vi "Main.vi"() -> ()   [LabVIEW 2013]
doc: "This template is for the Queued Message Handler design pattern.\n\nThe Event Handling Loop generates messages based on user interface actions.\n\nThe Message Handling Loop processes messages generated by the Event Handling Loop, or by other messages. The messages are string values, so new messages can be added easily to the Message Cases case structure in the Message Handling Loop. Each message cluster can also provide an optional value for Message Data, which is a variant that can be converted to whatever message-specific data is required."
uses:
  <vilib>/vision/Image Controls.llb/IMAQ Image.ctl
  <vilib>/vision/Avi.llb/IMAQ AVI2 Refnum.ctl
  Image Processing/Mask ROI FG Enum.ctl
  Message Passing/MsgQ Loops enum.ctl
  System Status/Status FG Enum.ctl
  Globals/Average Sector Data.vi
  controls/UI Data.ctl
  Message Queue/Message Queue.lvlib
  User Event - Stop/User Event - Stop.lvlib
  FPGA/FPGA Frame Grabbing.lvlib
  Image Processing/Image Processing.lvlib
  Common/State Machines/State Machine Lib.lvlib
  Message Passing/Main MsgQ.lvlib
  Common/GUI/GUI.lvlib
  <vilib>/rvi/interface/nirviReadWriteControl/nirviReadWriteControl.xnode
  FGs/FPGA_Reference.ctl
  FPGA Bitfiles/WBA256SectorsSim_FPGATarget.lvbitx
  Common/Timing/Timing Lib.lvlib
  <vilib>/rvi/errors/niLvFpgaMergeErrorWithErrorCode.vi
  NiFpgaLv.dll
  <vilib>/rvi/errors/niLvFpgaAdjustHostInterfaceError.vi
panel:
  in  "Auto Acq Total":u16=400
  in  "Auto Acquire?":bool
  out "Auto Acq Count":u16=401
  out "Codec Chosen":string="Motion JPEG (NI Vision)"
  in  "Codec index":i32=4
  out "Installed Codecs":string[](array[string])=["Microsoft Video 1", "Intel IYUV codec", "Cinepak Codec by Radius", "FF Video Codec 1 (FFV1) (NI Vision)", "Motion JPEG (NI Vision)", "Y800 Uncompressed Grey Scale (NI Vision)", "YUV 4:2:0 Planar (NI Vision)"]
  out "Overlay Image":T1
  out "AVI Refnum":T2
  in  "AVI FPS":u32=200
  in  "Save to AVI?":bool
  out "Single Acq Count":u16=1
  out "Frames Acquired":u32=1
  in  "Disable Background Subtraction":bool
  out "Analysis Ticks":u32
  out "Accumulate Ticks":u32
  out "FPGA Display Image":T1(plugin-control)
  out "Right Wingbeat Avg Graph":u8[](graph)=[9, 2, 3, 6, 23, 29, 37, 22, 2, 3, 2, 2, 2, 2, 2, 2]
  in  "Start Serial Server":bool=TRUE
  out "Left Wingbeat Avg Graph":u8[](graph)=[21, 5, 10, 10, 22, 33, 35, 21, 2, 2, 2, 2, 2, 2, 1, 2]
  in  "Stop Charts":bool
  in  "Wing ROIs":T3
  out "FPGA image info":T6={"Image Type"=0, "Unit"=enum."Undefined", "X Resolution"=1200, "Y Resolution"=788, "X Step"=1.0, "Y Step"=1.0, "Image Name"="Acquired"} {"Image Type" items=["Grayscale (U8)", "Grayscale (I16)", "Grayscale (SGL)", "Complex (CSG)", "RGB (U32)", "HSL (U32)", "RGB (U64)", "Grayscale (U16)"]}
  in  "Stream?":bool
  out "FPGA Image":T1
  in  "Test Visual Response":bool
  in  "Test FPGA":bool
  out "Status Update":string="01/27/2014 11:29:43.522 :  Loading Simulation Images\r01/27/2014 11:29:43.809 :  Completed Loading Simulation Images\r01/27/2014 11:29:43.911 :  Camera Initialized\r"
  in  "Define Mask":bool
  in  "Acquire Image":bool
  in  "Stop":bool
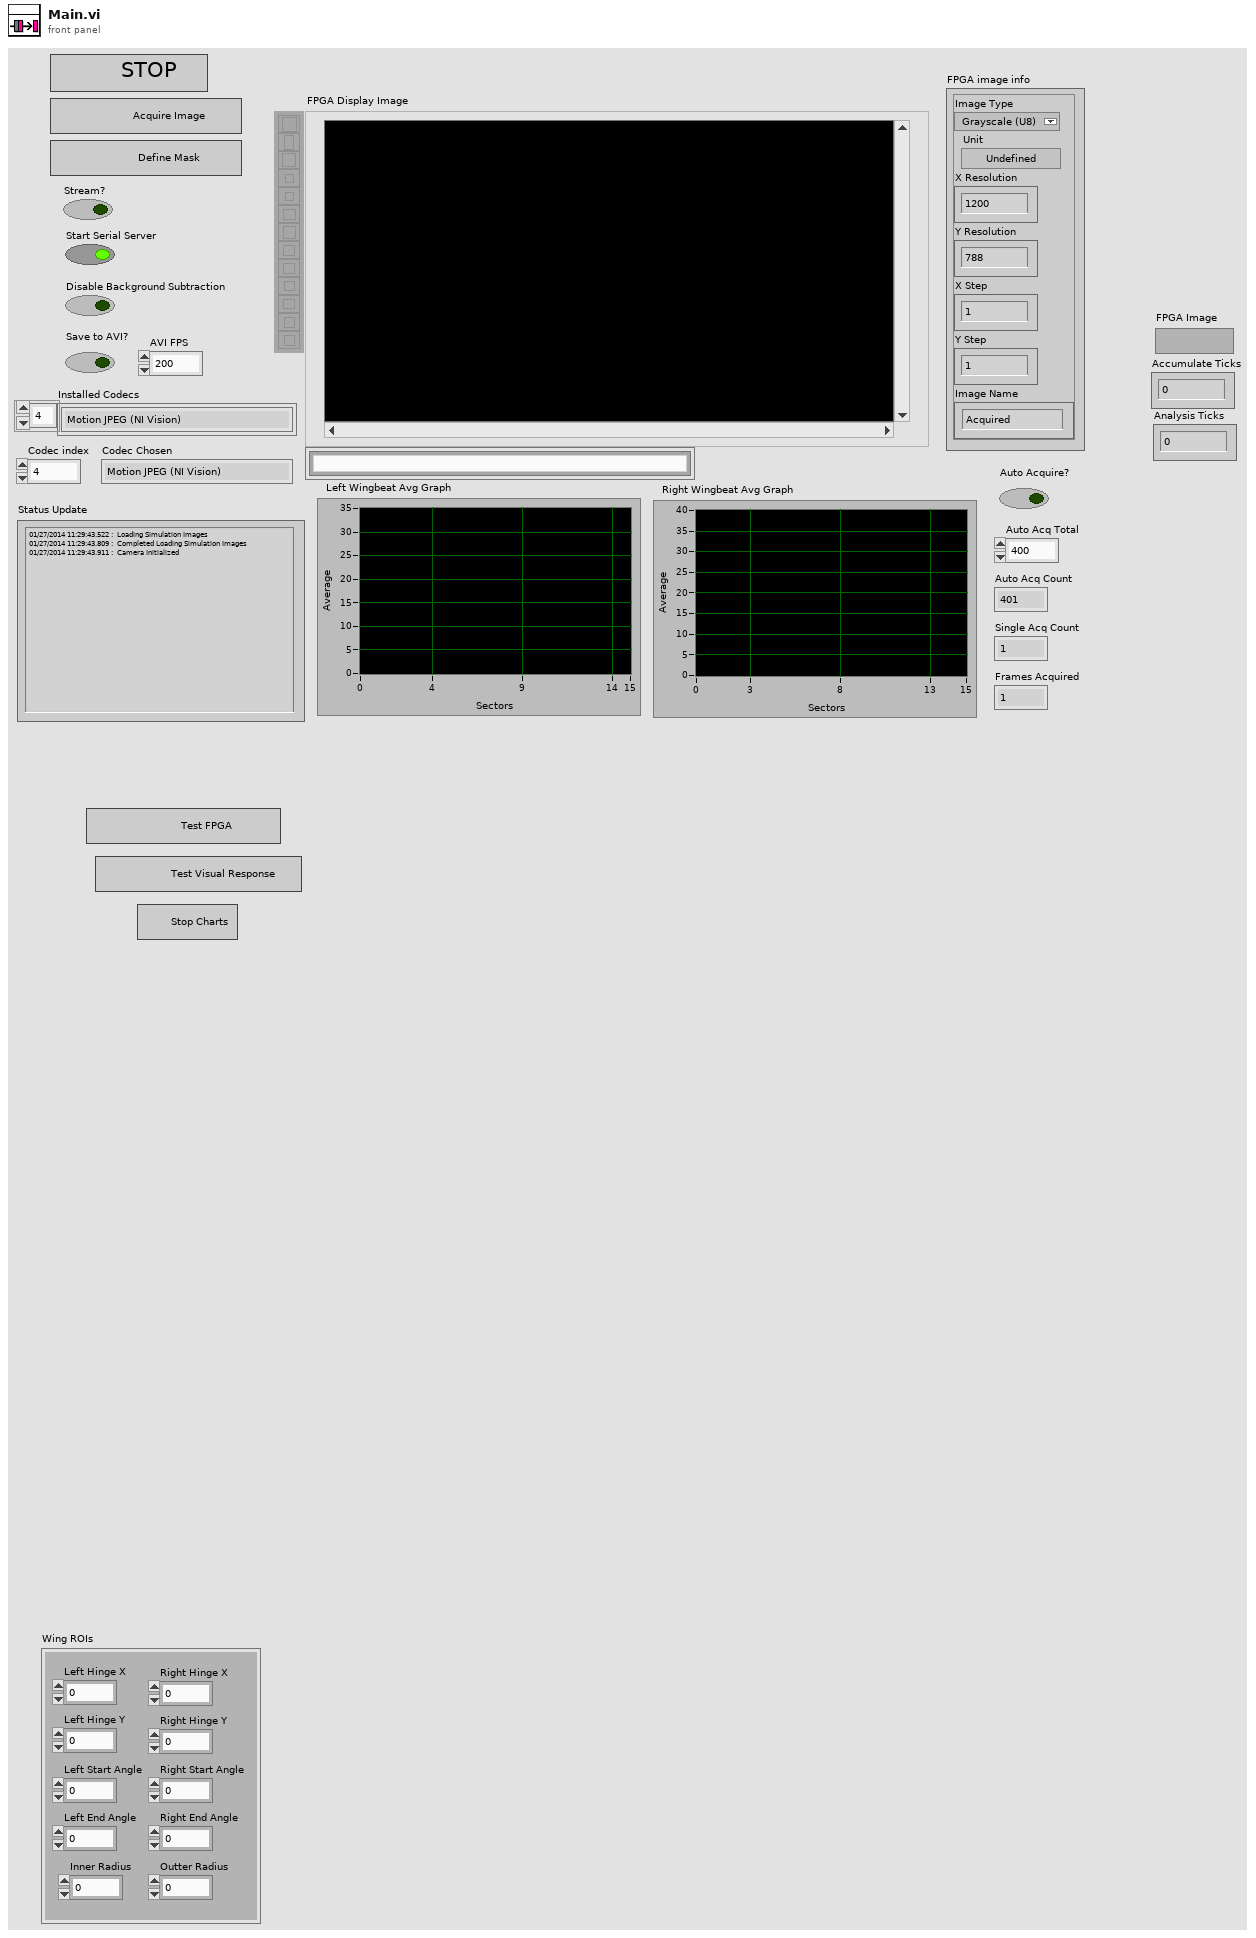
[diagram p1: front panel]
types:
  T1 = typedef "IMAQ Image.ctl" = refnum<image>
  T2 = typedef "IMAQ AVI2 Refnum.ctl" = refnum<k20>
  T3 = cluster{"Left Hinge X":u16, "Left Hinge Y":u16, "Inner Radius":u16, "Outter Radius":u16, "Right Hinge X":u16, "Right Hinge Y":u16, "Right Start Angle":i16, "Right End Angle":i16, "Left Start Angle":i16, "Left End Angle":i16}
  T4 = typedef "Image Type" = u32
  T5 = typedef "Image Unit" = enum32{"Undefined", "Angström", "Micrometer", "Millimeter", "Centimeter", "Meter", "Kilometer", "Microinch", "Inch", "Feet", "Nautical miles", "Standard miles", "Steps"}
  T6 = cluster{"Image Type":T4, "Unit":T5, "X Resolution":i32, "Y Resolution":i32, "X Step":sgl, "Y Step":sgl, "Image Name":string}
  T7 = typedef "State Machine Lib.lvlib/STATE cluster.ctl" = cluster{"State":string, "Parameters":variant}
  T8 = typedef "Main MsgQ.lvlib/MsgQ Loops enum.ctl" = enum16{"User Interface", "Image Acq"}
  T9 = typedef "Mask ROI FG Enum.ctl" = enum16{"Read", "Write", "Enable Background", "Disable Background"}
  T10 = typedef "Status FG Enum.ctl" = enum16{"Reset", "Read", "Write"}
  T11 = enum32{"Gray", "Binary", "Gradient", "Rainbow", "Temperature"}
  T12 = typedef "FPGA_Reference.ctl" = refnum<k20>
  T13 = typedef "Mask ROI Cluster.ctl" = cluster{"left annulus":T14, "right annulus":T14, "Threshold Range":cluster{"Lower value":dbl, "Upper value":dbl}, "[Avg BG]":u8[], "Number of Sectors":u8, "Left ROI":T15, "Right ROI":T15, "Left Start Angle Duty Cycle":fxp<+,8,0>, "Left End Angle Duty Cycle":fxp<+,8,0>, "Right End Angle Duty Cycle":fxp<+,8,0>, "Right Start Angle Duty Cycle":fxp<+,8,0>, "[Sector ROIs]":T15[]}
  T14 = typedef "IMAQ Circle" = cluster{"Center X":i32, "Center Y":i32, "Inner Radius":i32, "Outer Radius":i32, "Start Angle":dbl, "End Angle":dbl}
  T15 = typedef "ROI Descriptor" = cluster{"Global Rectangle":i32[], "Contours":cluster{"ID":enum32{"External", "Internal"}, "Type":u32, "Coordinates":i32[]}[]}
  T16 = typedef "UI Data.ctl" = cluster{"Boolean <Replace Me>":bool, "Initial Message":string, "Numeric <Replace Me>":dbl, "Acquire Image Ref":refnum<vi>, "Define Mask Ref":refnum<vi>, "Status Update Ref":refnum<vi>, "Stop Button Ref":refnum<vi>, "FPGA Image":T1, "Processed Image":T1, "Left Annulus":cluster{"Center X":i32, "Center Y":i32, "Inner Radius":i32, "Outer Radius":i32, "Start Angle":dbl, "End Angle":dbl}, "Right Annulus":cluster{"Center X":i32, "Center Y":i32, "Inner Radius":i32, "Outer Radius":i32, "Start Angle":dbl, "End Angle":dbl}}
  T17 = typedef "Message Queue.lvlib/All Message Queues.ctl" = cluster{"UI":refnum<queue>}
  T18 = cluster{"Center X":i32, "Center Y":i32, "Inner Radius":i32, "Outer Radius":i32, "Start Angle":dbl, "End Angle":dbl}
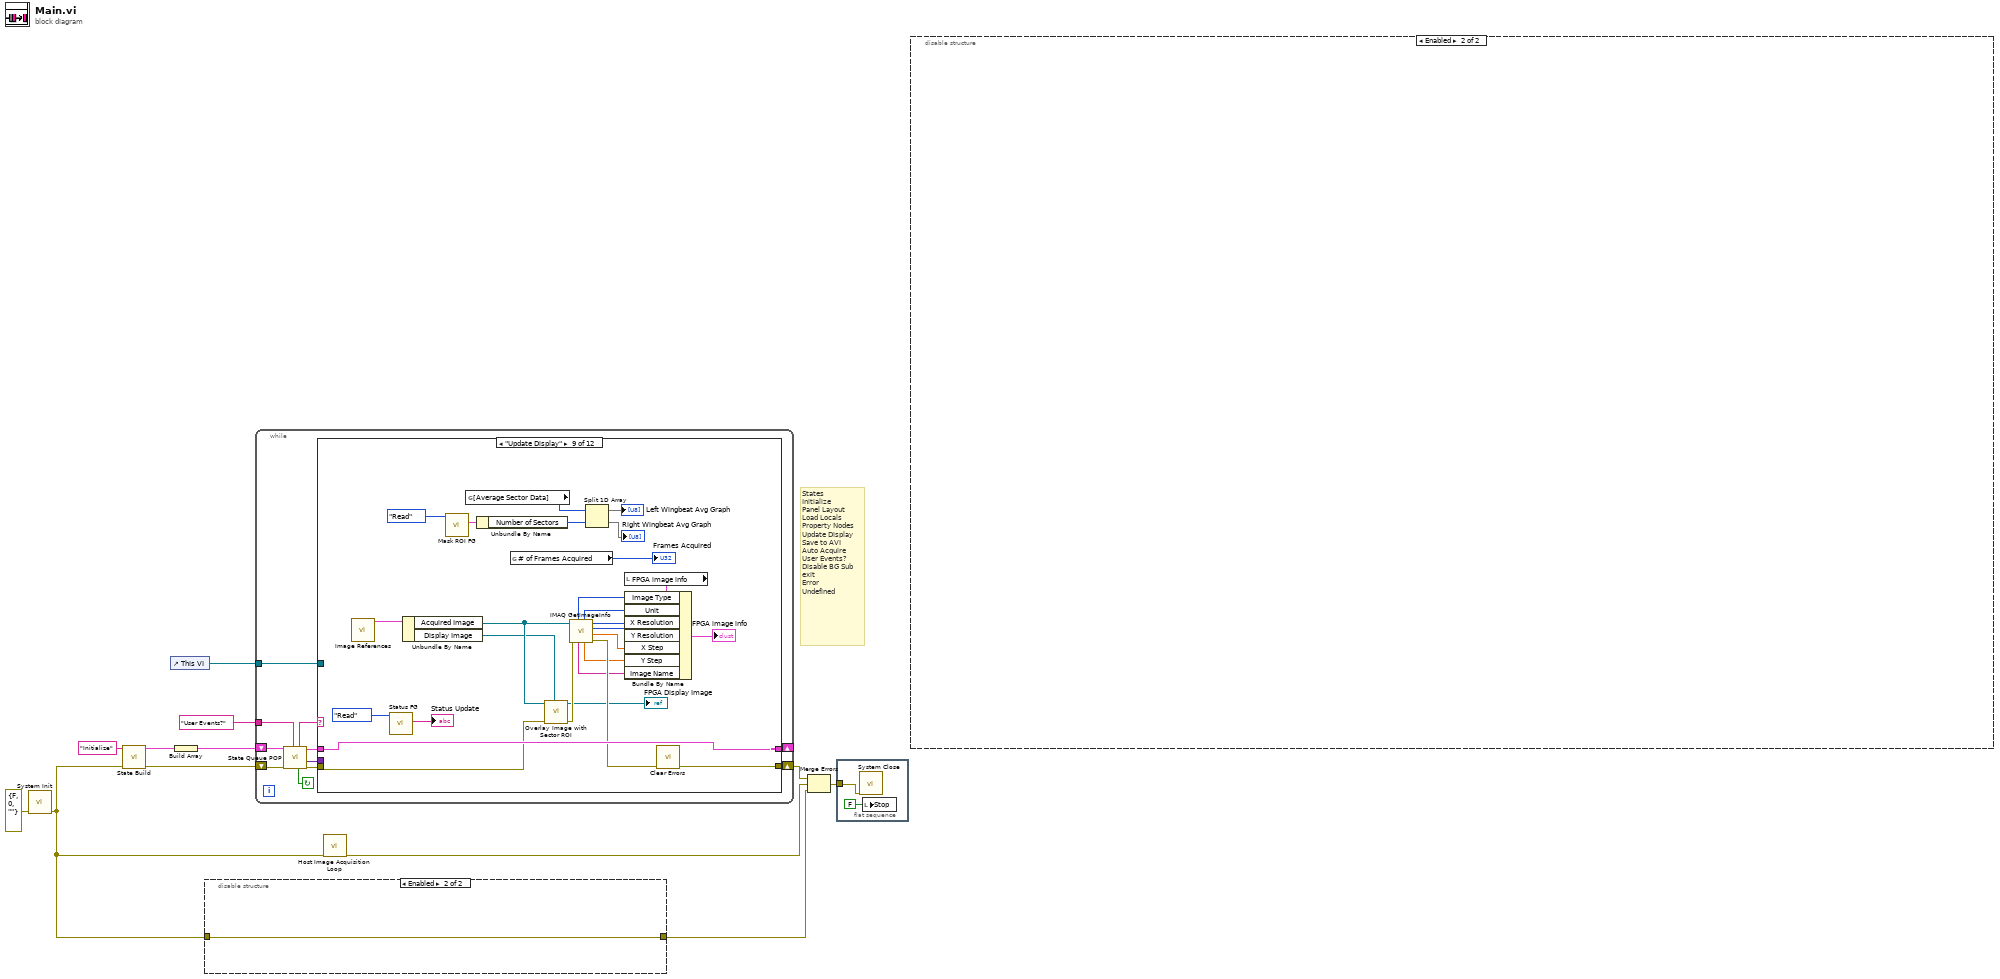
[diagram p0: block diagram]
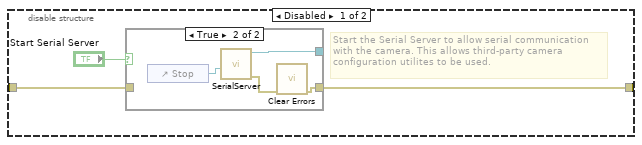
[diagram p2: hidden frame]
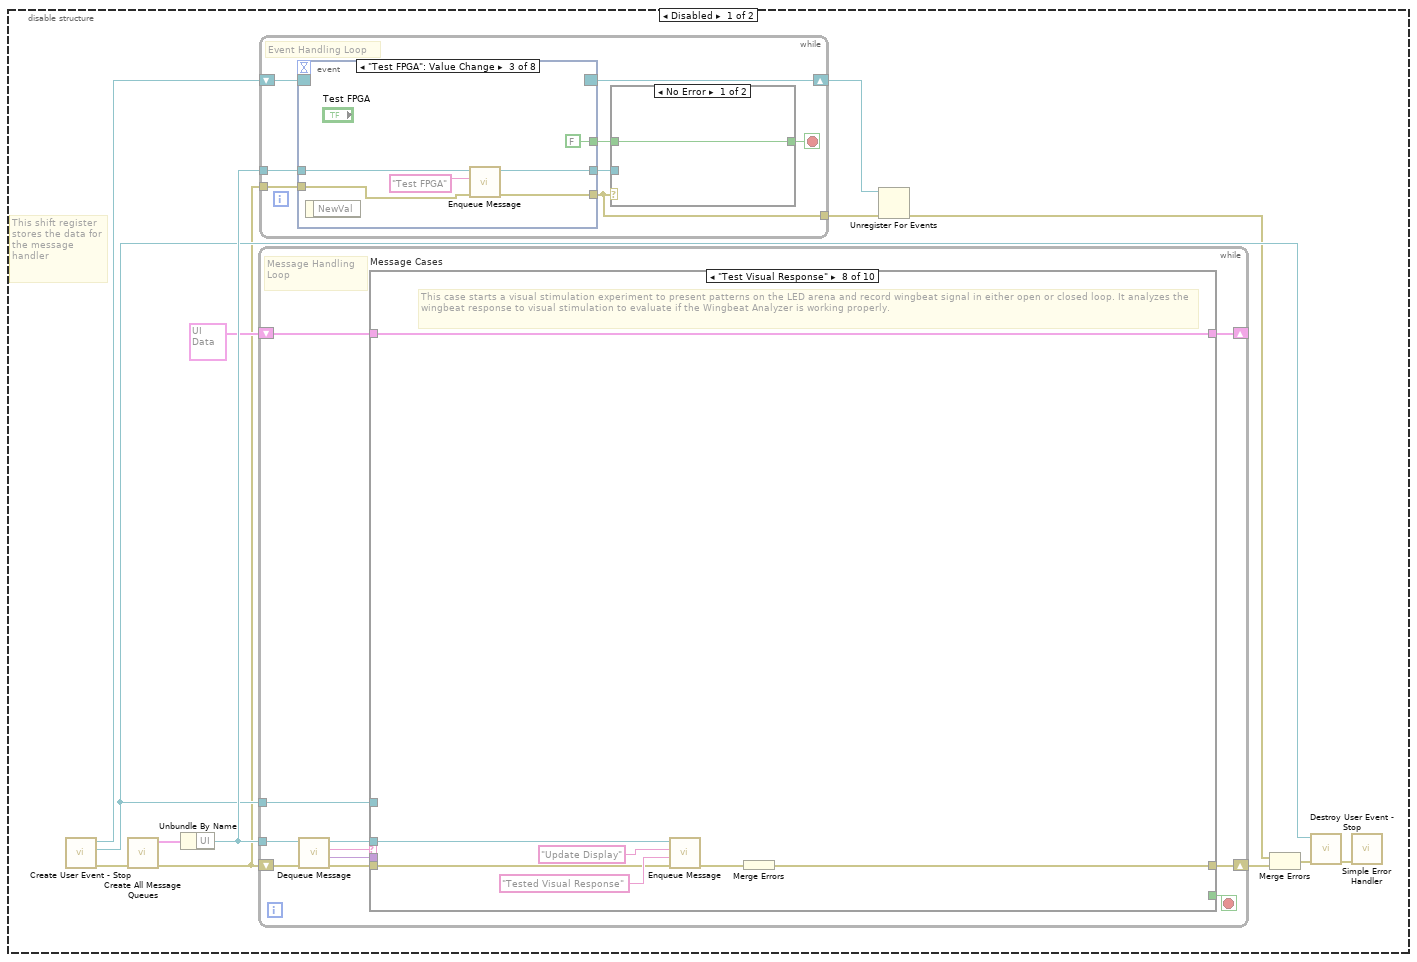
[diagram p4: hidden frame]
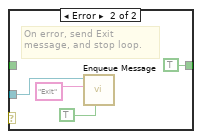
[diagram p5: hidden frame]
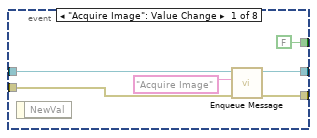
[diagram p6: hidden frame]
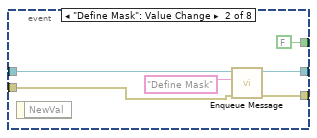
[diagram p7: hidden frame]
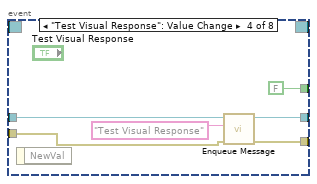
[diagram p8: hidden frame]
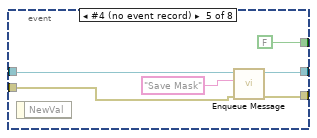
[diagram p9: hidden frame]
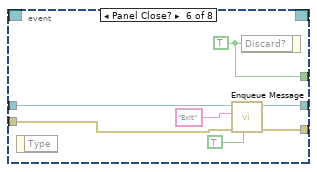
[diagram p10: hidden frame]
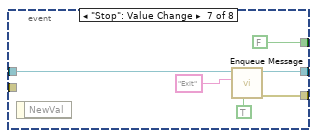
[diagram p11: hidden frame]
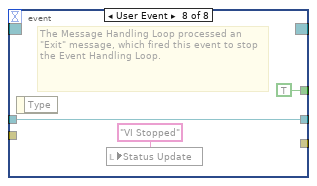
[diagram p12: hidden frame]
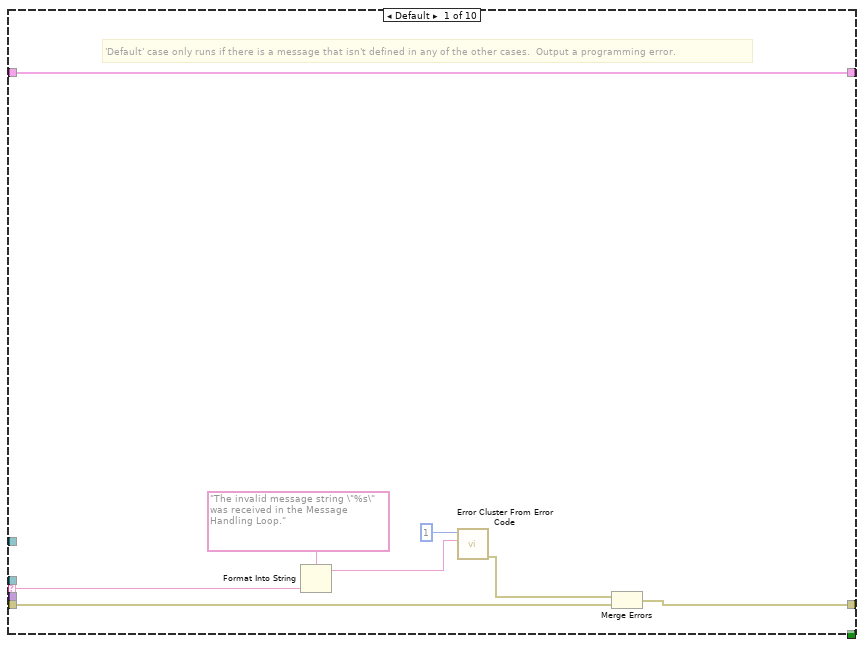
[diagram p13: hidden frame]
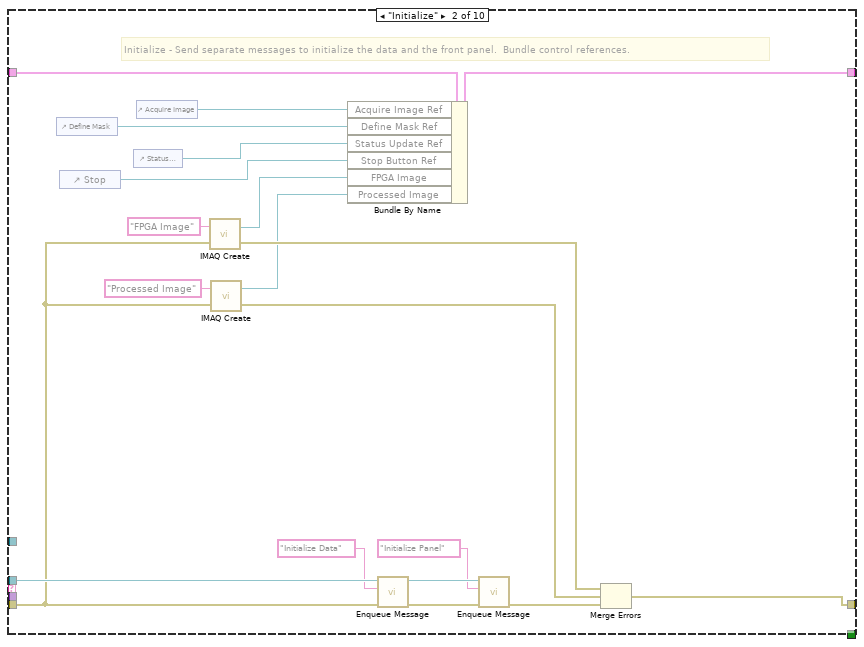
[diagram p14: hidden frame]
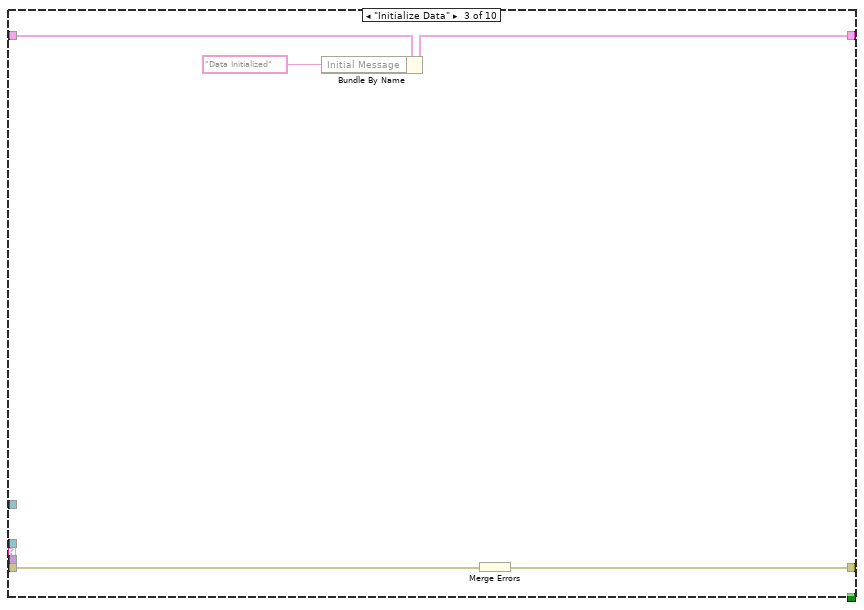
[diagram p15: hidden frame]
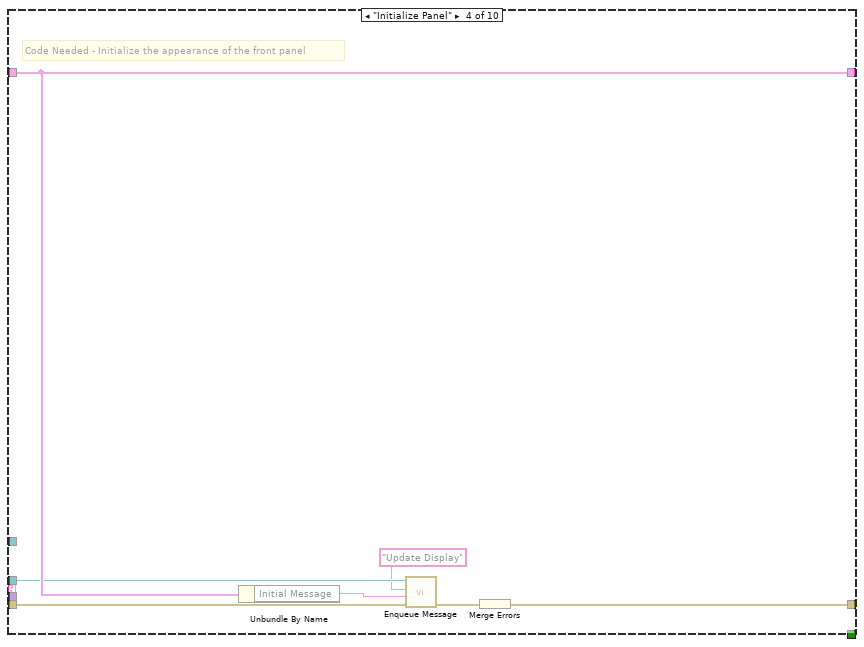
[diagram p16: hidden frame]
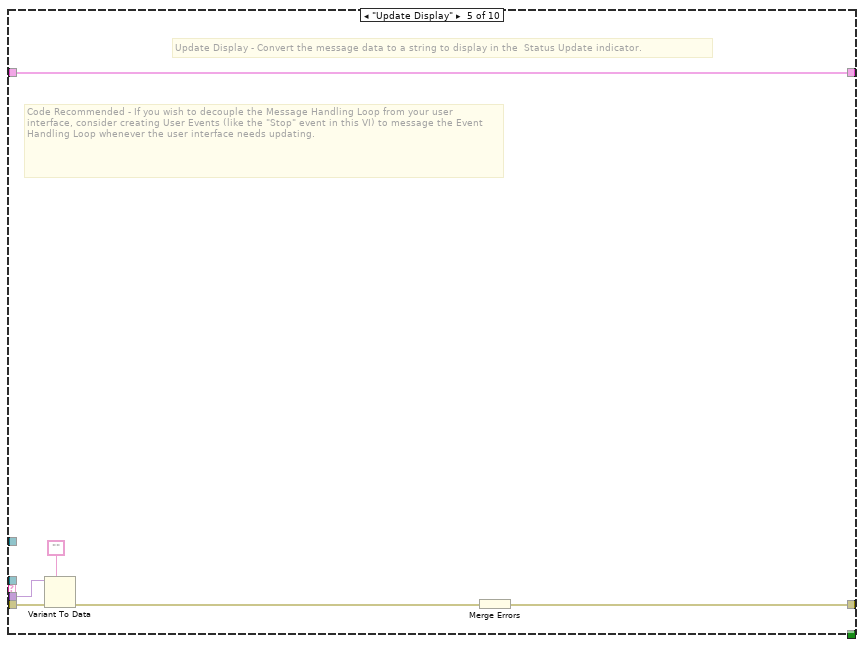
[diagram p17: hidden frame]
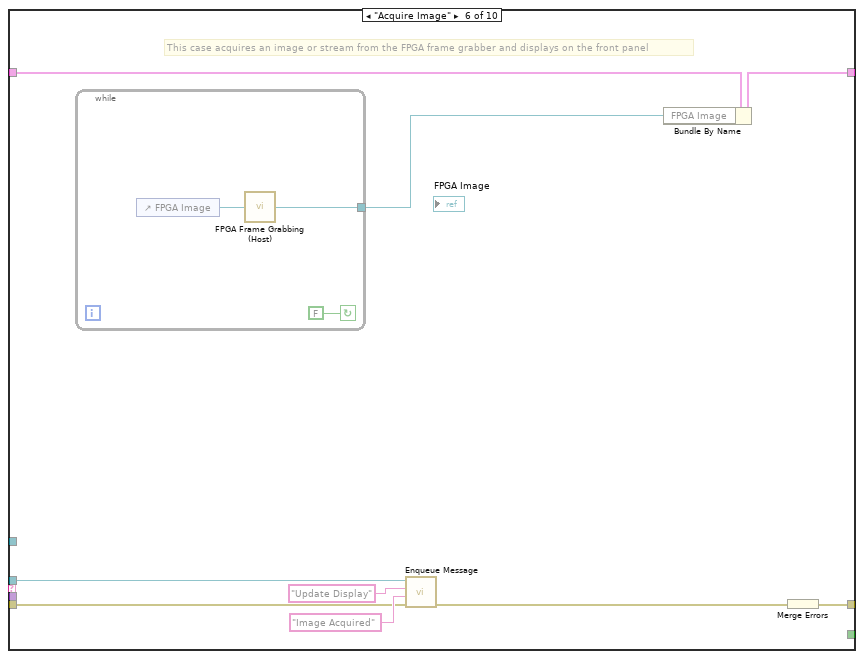
[diagram p18: hidden frame]
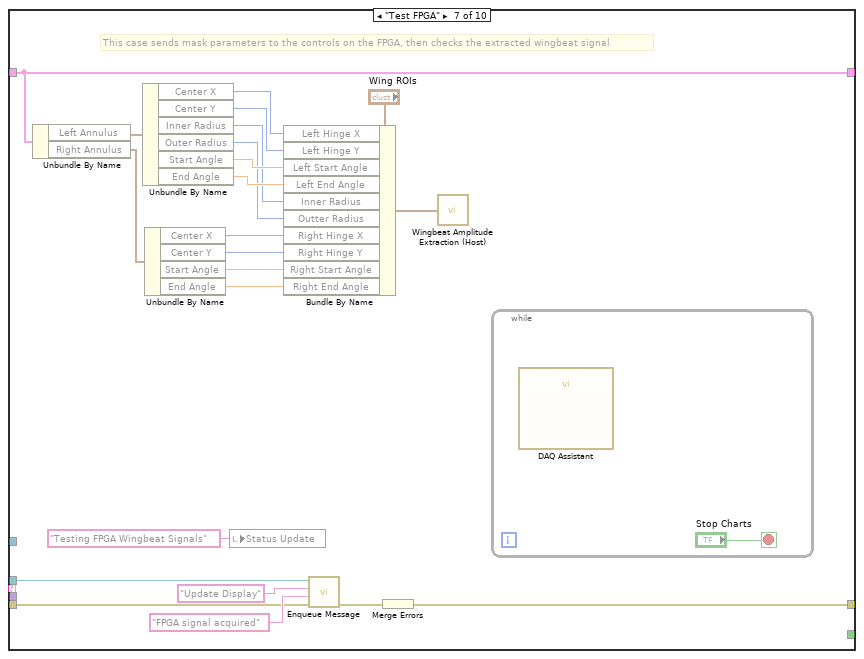
[diagram p19: hidden frame]
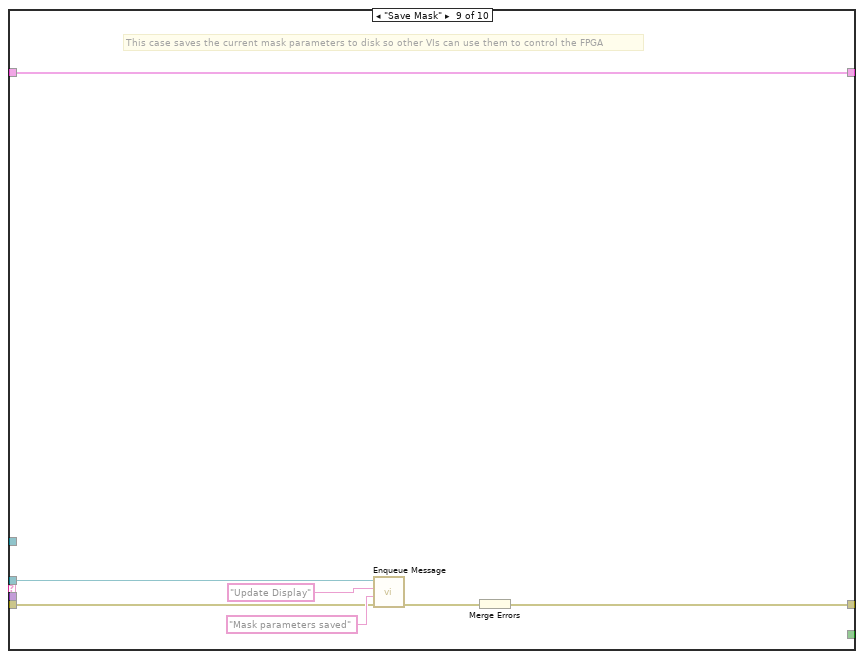
[diagram p20: hidden frame]
diagram:
  # "States\nInitialize\nPanel Layout\nLoad Locals\nProperty Nodes\nUpdate Display\nSave to AVI\nAuto Acquire\nUser Events?\nDisable BG Sub\nexit\nError\nUndefined"
  n1 = call "System Init.vi"("error in (no error)"=errorcluster {"status"=FALSE, "code"=0, "source"=""}) -> ("error out"=w11:errorcluster)  [unwired: 10 in]
  n2 = call "State Build.vi"("error in (no error)"=w11, "State"="Initialize") -> ("error out"=w7:errorcluster, "State Out"=w9:T7)  [unwired: 8 in]
  n3 = control-ref of="This VI"() -> (w5:refnum<vi>)
  n4 = Build Array(w9) -> (w8:T7[])
  n5 = disable-structure shown="Enabled" {
    disable-tunnel: w11 -> [w14 w21]
    disable-tunnel: [w13 w21] -> w1
    frame Disabled {
      # "Start the Serial Server to allow serial communication\nwith the camera. This allows third-party camera\nconfiguration utilites to be used."
      n6 = case shown="True" "Start Serial Server" {
        tunnel: [_ w20] -> _
        tunnel: w14 -> [w16 _]
        tunnel: [w16 w18] -> w13
        frame False {
        }
        frame True {
          n7 = control-ref of="Stop"() -> (w19:refnum<vi>)
          n8 = call "SerialServer.vi"("Stop Refnum"=w19) -> ("error out"=w17:errorcluster, "FPGA VI Reference Out"=w20:refnum<k20>)  [unwired: 5 in]
          n9 = call <vilib>:"Clear Errors.vi"("error in (no error)"=w17) -> ("error out"=w18:errorcluster)  [unwired: 6 in]
        }
      }
    }
    frame Enabled {
    }
  }
  n10 = while {
    shift-right: [w26] -> _
    shift-left: w8 -> [w32]
    shift-right: [w24] -> w4
    shift-left: w7 -> [w31]
    tunnel: "User Events?" ("State") -> [w29]
    tunnel: w5 -> [w27]
    stop <- w30 continue-if-true
    n11 = call "State Queue POP.vi"("Default state"=w29, "error in (no error)"=w31, "State que in"=w32) -> ("error out"=w23:errorcluster, "Parameters"=w22:variant, "State que out"=w25:T7[], "Not Exit?"=w30:bool, "State case out"=w28:string)  [unwired: 4 in]
    n12 = case shown="\"Update Display\"" w28 {
      tunnel: w27 -> [_ _ w43 _ _ _ _ _ _ _ _ _]
      tunnel: [w34 w35 w40 w50 w71 w76 w77 w94 w177 w182 w194 w227] -> w26
      tunnel: w25 -> [w34 w38 w40 w50 w71 w76 w77 w93 w177 w182 w196 _]
      tunnel: [w33 w36 w41 w45 w70 w74 w78 w92 w175 w183 w195 w220] -> w24
      tunnel: w23 -> [w33 w37 w42 w46 w70 w75 w89 w91 w159 w179 w197 w224]
      tunnel: w22 -> [_ _ _ _ _ _ w88 w90 _ _ _ _]
      frame Default {
      }
      frame "Initialize" {
        n13 = call "State Queue PUSH multiple states no parameters.vi"("States to queue"=string[] ["Panel Layout", "Load Locals", "Property Nodes", "Update Display"], "error in (no error)"=w37, "State que in"=w38) -> ("error out"=w36:errorcluster, "State que out"=w35:T7[])  [unwired: 7 in]
      }
      frame "Panel Layout" {
        # "Reset origin to 0,0"
        n14 = call "Reset all pane origins.vi"("error in (no error"=w42, "Vi Ref In"=w43) -> ("error out"=w41:errorcluster)  [unwired: 8 in, 1 out]
      }
      frame "Load Locals" {
        w44 = u16 0
        w49 = FALSE ("Stream?")
        n15 = local write "Stream?"(w49) -> ()
        n16 = local write "Disable Background Subtraction"(w49) -> ()
        n17 = case shown="True" "Save to AVI?" {
          tunnel: w46 -> [w51 w53]
          tunnel: [w51 w58] -> w47
          frame False {
          }
          frame True {
            w62 = T4 4 items=["Grayscale (U8)", "Grayscale (I16)", "Grayscale (SGL)", "Complex (CSG)", "RGB (U32)", "HSL (U32)", "RGB (U64)", "Grayscale (U16)"] ("Image Type")
            n18 = Current VI's Path() -> (path=w69:path)
            n19 = call "IMAQ Create"("Image Name"="Overlay Image", "Image Type"=w62, "error in (no error)"=w53) -> ("New Image"=w54:T1, "error out"=w59:errorcluster)  [unwired: 2 in]
            "Overlay Image" <- w54
            n20 = call "File Dialog"("start path"=w69, "prompt"="Specify AVI Name to Save", "error in"=w53, "pattern (all files)"="*.avi") -> ("selected path"=w66:path, "error out"=w61:errorcluster)  [unwired: 8 in, 2 out]
            n21 = call "IMAQ AVI2 Get Codec Names"("error in (no error)"=w53, "Image"=w54) -> ("error out"=w52:errorcluster, "Codec Names"=w57:string[])  [unwired: 8 in]
            "Installed Codecs" <- w57
            n22 = Index Array(array=w57, index="Codec index") -> (element=w55:string)
            "Codec Chosen" <- w55
            n23 = call "IMAQ AVI2 Create"("error in (no error)"=w61, "Codec"=w55, "Frames Per Second"="AVI FPS", "AVI Path"=w66) -> ("error out"=w60:errorcluster, "AVI Refnum"=→"AVI Refnum":T2)  [unwired: 6 in]
            n24 = Merge Errors(w60, w59, w52) -> (w58:errorcluster)
          }
        }
        n25 = local write "Auto Acq Count"(w44) -> ()
        n26 = local write "Single Acq Count"(w44) -> ()
        n27 = local write "Frames Acquired"(w44) -> ()
        n28 = Merge Errors(w47, w46) -> (w45:errorcluster)
      }
      frame "Property Nodes" {
      }
      frame "Define Mask" {
        n29 = call "Image References.vi"() -> ("Images"=w73:cluster{"Acquired Image":T1, "Display Image":T1})  [unwired: 10 in, 1 out]
        n30 = Unbundle By Name(w73) -> ("Acquired Image"=w72:T1)
        n31 = call "Define Mask.vi"("error in (no error)"=w75, "FPGA Image"=w72) -> ("error out"=w74:errorcluster)  [unwired: 9 in]
      }
      frame "Disable BG Sub" {
        n32 = Variant To Data(error in=w89, type=FALSE, Variant=w88) -> (data=w86:bool, error out=w83:errorcluster)
        n33 = Select(t=Mask_ROI_FG_Enum."Disable Background" ("Operation"), s=w86, f=Mask_ROI_FG_Enum."Enable Background" ("Operation")) -> (s? t:f=w82:T9)
        n34 = call "Mask ROI FG.vi"("error in (no error)"=w83, "Operation"=w82) -> ("error out"=w79:errorcluster)  [unwired: 8 in, 1 out]
        n35 = call "Send MsgQ.vi"("error in (no error)"=w79, "Message String"="Update Sector Parameters", "Send to MsgQ"=MsgQ_Loops_enum."Image Acq") -> ("error out"=w78:errorcluster)  [unwired: 8 in]
      }
      frame "User Events?" {
        n36 = event shown="[0] Timeout" {
          selector: _ -> [_ _ _ _ _ _ _]
          dyn-events: _ -> [_ _ _ _ _ _ _]
          timeout: 200 -> [_ _ _ _ _ _ _]
          tunnel: [w97 w108 w125 w130 w137 w143 w146] -> w94
          tunnel: w93 -> [w98 w109 w128 w130 w139 w145 w149]
          tunnel: [w99 w107 w126 w131 w136 w142 w147] -> w92
          tunnel: w91 -> [w100 w110 w127 w132 w138 w144 w148]
          tunnel: w90 -> [_ _ _ _ _ _ _]
          event Timeout {
            n37 = event-data() -> ()  [unwired: 1 in, 3 out]
            n38 = disable-structure shown="Enabled" {
              frame Disabled {
                n39 = call "FPGA Reference FG.vi"() -> ("FPGA VI Reference Out"=w103:T12)  [unwired: 11 in]
                n40 = xnode "Read/Write Control"("FPGA VI Reference In"=w103) -> ("Accumulate Ticks"=→"Accumulate Ticks", "Analysis Ticks"=→"Analysis Ticks":u32)  [unwired: 1 in, 2 out]
              }
              frame Enabled {
              }
            }
            n41 = call "State Queue PUSH.vi"("State case"="Update Display", "error in (no error)"=w100, "State que in"=w98) -> ("error out"=w99:errorcluster, "State que out"=w97:T7[])  [unwired: 7 in]
          }
          event "Acquire Image": Value Change {
            n42 = event-data() -> ()  [unwired: 1 in, 6 out]
            n43 = local read "Save to AVI?"() -> (w111:bool)
            n44 = call "Send MsgQ.vi"("error in (no error)"=w110, "Message String"="Acquire Single Image", "Send to MsgQ"=MsgQ_Loops_enum."Image Acq") -> ("error out"=w106:errorcluster)  [unwired: 8 in]
            n45 = call "Wait (ms) with error IO.vi"("error in (no error)"=w106, "milliseconds to wait"=u32 500) -> ("error out"=w105:errorcluster)  [unwired: 3 in]
            n46 = case shown="True" w111 {
              tunnel: w109 -> [w118 w122]
              tunnel: w105 -> [w117 w121]
              tunnel: [w118 w120] -> w108
              tunnel: [w117 w119] -> w107
              frame False {
              }
              frame True {
                n47 = call "State Queue PUSH multiple states no parameters.vi"("States to queue"=string[] ["Update Display", "Save to AVI", "", ""], "error in (no error)"=w121, "State que in"=w122) -> ("error out"=w119:errorcluster, "State que out"=w120:T7[])  [unwired: 7 in]
              }
            }
            n48 = feedback #1(u16 0 ("Frame Count")) -> (w113:u16)
            n49 = Increment(x=w113) -> (x+1=w112:u16)
            "Single Acq Count" <- w112
            n50 = feedback-in #1(w112) -> ()
          }
          event "Auto Acquire?": Value Change {
            n51 = event-data() -> ()  [unwired: 1 in, 6 out]
            n52 = call "State Queue PUSH multiple states no parameters.vi"("States to queue"=string[] ["Auto Acquire"], "error in (no error)"=w127, "State que in"=w128) -> ("error out"=w126:errorcluster, "State que out"=w125:T7[])  [unwired: 7 in]
          }
          event "Stream?": Value Change {
            n53 = event-data() -> ("NewVal"=w129:bool)  [unwired: 1 in, 5 out]
            n54 = call "Send MsgQ.vi"("error in (no error)"=w132, "Data In"=w129, "Message String"="Stream Image", "Send to MsgQ"=MsgQ_Loops_enum."Image Acq") -> ("error out"=w131:errorcluster)  [unwired: 7 in]
          }
          event "Define Mask": Value Change {
            n55 = event-data() -> ()  [unwired: 1 in, 6 out]
            n56 = call "State Queue PUSH.vi"("State case"="Define Mask", "error in (no error)"=w138, "State que in"=w139) -> ("error out"=w136:errorcluster, "State que out"=w137:T7[])  [unwired: 7 in]
          }
          event "Disable Background Subtraction": Value Change {
            n57 = event-data() -> ("NewVal"=w140:bool)  [unwired: 1 in, 5 out]
            n58 = call "State Queue PUSH.vi"("State case"="Disable BG Sub", "error in (no error)"=w144, "Parameters"=w140, "State que in"=w145) -> ("error out"=w142:errorcluster, "State que out"=w143:T7[])  [unwired: 6 in]
          }
          event "Stop": Value Change {
            n59 = event-data() -> ()  [unwired: 1 in, 6 out]
            n60 = call "State Queue PUSH.vi"("State case"="exit", "error in (no error)"=w148, "State que in"=w149) -> ("error out"=w147:errorcluster, "State que out"=w146:T7[])  [unwired: 7 in]
          }
        }
      }
      frame "Update Display" {
        n61 = call "Image References.vi"() -> ("Images"=w155:cluster{"Acquired Image":T1, "Display Image":T1})  [unwired: 10 in, 1 out]
        n62 = call "Status FG.vi"("Operation"=Status_FG_Enum."Read") -> ("Status Out"=→"Status Update":string)  [unwired: 9 in, 1 out]
        n63 = Unbundle By Name(w155) -> ("Acquired Image"=w154:T1, "Display Image"=w153:T1)
        n64 = call "Mask ROI FG.vi"("Operation"=Mask_ROI_FG_Enum."Read") -> ("Mask ROI Out"=w172:T13)  [unwired: 9 in, 1 out]
        n65 = global read "Average Sector Data.vi" "[Average Sector Data]"() -> (w174:u8[])
        n66 = Unbundle By Name(w172) -> ("Number of Sectors"=w169:u8)
        n67 = global read "Average Sector Data.vi" "# of Frames Acquired"() -> (→"Frames Acquired":u32)
        n68 = call "Overlay Image with Sector ROI.vi"("FPGA Display Image In"=w153, "error in"=w159, "FPGA Image"=w154) -> ("error out"=w158:errorcluster, "FPGA Display Image Out"=→"FPGA Display Image":T1)  [unwired: 7 in]
        n69 = call "IMAQ GetImageInfo"("error in (no error)"=w158, "Image"=w154) -> ("error out"=w176:errorcluster, "X Step"=w164:sgl, "Y Resolution"=w163:i32, "X Resolution"=w162:i32, "Y Step"=w165:sgl, "Unit"=w161:T5, "Image Name"=w166:string, "Image Type"=w160:T4)  [unwired: 2 in]
        n70 = Split 1D Array(array=w174, index=w169) -> (first subarray=→"Left Wingbeat Avg Graph":u8[], second subarray=→"Right Wingbeat Avg Graph":u8[])
        n71 = local read "FPGA image info"() -> (w168:T6)
        n72 = Bundle By Name(cluster=w168, "Image Type"=w160, "Unit"=w161, "X Resolution"=w162, "Y Resolution"=w163, "X Step"=w164, "Y Step"=w165, "Image Name"=w166) -> (→"FPGA image info":T6)
        n73 = call <vilib>:"Clear Errors.vi"("error in (no error)"=w176) -> ("error out"=w175:errorcluster)  [unwired: 6 in]
      }
      frame "Save to AVI" {
        n74 = local read "Overlay Image"() -> (w184:T1)
        n75 = local read "FPGA Display Image"() -> (w188:T1)
        n76 = call "IMAQ GetPalette"("Palette Number (gray)"=T11."Gradient", "error in (no error)"=w179) -> ("Color Palette"=w180:cluster{"Red":u8, "Green":u8, "Blue":u8}[], "error out"=w178:errorcluster)  [unwired: 3 in]
        n77 = local read "AVI Refnum"() -> (w185:T2)
        n78 = call "IMAQ Merge Overlay"("error in (no error)"=w178, "Color Palette"=w180, "Image Dst"=w184, "Image Src"=w188) -> ("error out"=w186:errorcluster, "Image Dst Out"=w187:T1)  [unwired: 6 in]
        n79 = call "IMAQ AVI2 Write Frame"("error in (no error)"=w186, "Image"=w187, "AVI Refnum"=w185) -> ("error out"=w183:errorcluster)  [unwired: 6 in, 2 out]
      }
      frame "Auto Acquire" {
        n80 = feedback #2(u16 0 ("Frame Count")) -> (w192:u16)
        n81 = Increment(x=w192) -> (x+1=w189:u16)
        "Auto Acq Count" <- w189
        n82 = Greater?(x=w189, y="Auto Acq Total") -> (0:w191:bool)
        n83 = feedback-in #2(w189) -> ()
        n84 = case shown="True" w191 {
          tunnel: w197 -> [w201 w218]
          tunnel: w196 -> [w200 w219]
          tunnel: [w199 w218] -> w195
          tunnel: [w198 w219] -> w194
          frame False {
            n85 = call "Send MsgQ.vi"("error in (no error)"=w201, "Message String"="Acquire Single Image", "Send to MsgQ"=MsgQ_Loops_enum."Image Acq") -> ("error out"=w204:errorcluster)  [unwired: 8 in]
            n86 = local read "Save to AVI?"() -> (w205:bool)
            n87 = call "Wait (ms) with error IO.vi"("error in (no error)"=w204, "milliseconds to wait"=u32 500) -> ("error out"=w203:errorcluster)  [unwired: 3 in]
            n88 = case shown="True" w205 {
              tunnel: w200 -> [w212 w216]
              tunnel: w203 -> [w211 w215]
              tunnel: [w210 w214] -> w198
              tunnel: [w209 w213] -> w199
              frame False {
                n89 = call "State Queue PUSH multiple states no parameters.vi"("States to queue"=string[] ["Update Display", "Auto Acquire"], "error in (no error)"=w211, "State que in"=w212) -> ("error out"=w209:errorcluster, "State que out"=w210:T7[])  [unwired: 7 in]
              }
              frame True {
                n90 = call "State Queue PUSH multiple states no parameters.vi"("States to queue"=string[] ["Update Display", "Save to AVI", "Auto Acquire", ""], "error in (no error)"=w215, "State que in"=w216) -> ("error out"=w213:errorcluster, "State que out"=w214:T7[])  [unwired: 7 in]
              }
            }
          }
          frame True {
          }
        }
      }
      frame "exit" {
        n91 = local read "Save to AVI?"() -> (w226:bool)
        n92 = case shown="True" w226 {
          tunnel: w224 -> [w228 w230]
          tunnel: [w228 w229] -> w223
          frame False {
          }
          frame True {
            n93 = local read "AVI Refnum"() -> (w231:T2)
            n94 = call "IMAQ AVI2 Close"("error in (no error)"=w230, "AVI Refnum"=w231) -> ("error out"=w229:errorcluster)  [unwired: 9 in]
          }
        }
        n95 = call "Broadcast Exit.vi"("error in"=w224) -> ("error out"=w221:errorcluster)  [unwired: 10 in]
        n96 = call "IMAQ Dispose"("All Images? (No)"=TRUE, "error in (no error)"=w224) -> ("error out"=w222:errorcluster)  [unwired: 4 in]
        n97 = Merge Errors(w223, w222, w221) -> (w220:errorcluster)
        n98 = call "Queue EXIT state.vi"() -> ("Exit State Q"=w227:T7[])  [unwired: 1 in]
      }
    }
  }
  n99 = call "Host Image Acquisition Loop.vi"("error in"=w11) -> ("error out"=w3:errorcluster)  [unwired: 10 in]
  n100 = Merge Errors(w4, w3, w1) -> (w2:errorcluster)
  n101 = flat-sequence {
    tunnel: w2 -> [w233]
    frame #0 {
      n102 = call "System Close.vi"("error in (no error)"=w233) -> ()  [unwired: 10 in, 1 out]
      n103 = local write "Stop"(FALSE ("Stop")) -> ()
    }
  }
  n104 = disable-structure shown="Enabled" {
    frame Disabled {
      # "This shift register\nstores the data for the message handler"
      n105 = call "Create User Event - Stop.vi"() -> ("error out"=w242:errorcluster, "User Event - Stop"=w239:refnum<user-event>, "Stop Event Registration Refnum"=w243:refnum<event-registration>)  [unwired: 9 in]
      n106 = call "Create All Message Queues.vi"("error in (no error)"=w242) -> ("error out"=w234:errorcluster, "Message Queues out"=w246:T17)  [unwired: 9 in]
      n107 = Unbundle By Name(w246) -> ("UI"=w244:refnum<queue>)
      n108 = while {
        tunnel: w244 -> [w306]
        shift-right: [w315] -> _
        shift-left: T16 {"Boolean <Replace Me>"=TRUE, "Initial Message"="", "Numeric <Replace Me>"=0.0, "Acquire Image Ref"=refnum, "Define Mask Ref"=refnum, "Status Update Ref"=refnum, "Stop Button Ref"=refnum, "FPGA Image"=refnum, "Processed Image"=refnum, "Left Annulus"={"Center X"=0, "Center Y"=0, "Inner Radius"=0, "Outer Radius"=0, "Start Angle"=0.0, "End Angle"=0.0}, "Right Annulus"={"Center X"=0, "Center Y"=0, "Inner Radius"=0, "Outer Radius"=0, "Start Angle"=0.0, "End Angle"=0.0}} ("Data Cluster") -> [w316]
        tunnel: w239 -> [w312]
        shift-right: [w313] -> w245
        shift-left: w234 -> [w311]
        stop <- w314 stop-if-true
        # "Message Handling Loop"
        n109 = call "Dequeue Message.vi"("error in (no error)"=w311, "Message Queue"=w306) -> ("error out"=w310:errorcluster, "Message Data"=w308:variant, "Message"=w309:string, "dup Message Queue"=w307:refnum<queue>)  [unwired: 6 in]
        n110 = case "Message Cases" shown="\"Test Visual Response\"" w309 {
          selector: w309 -> [w322 _ _ _ _ _ _ _ _ _]
          tunnel: w307 -> [_ w342 _ w353 _ w370 w393 w401 w409 w425]
          tunnel: w310 -> [w319 w327 w349 w354 w361 w365 w394 w402 w407 w414]
          tunnel: [w317 w329 w345 w355 w362 w372 w392 w400 w412 w421] -> w313
          tunnel: w316 -> [w324 w339 w348 w356 w363 w367 w391 w406 w413 w424]
          tunnel: [w324 w338 w347 w356 w363 w366 w391 w406 w413 w424] -> w315
          tunnel: [_ _ _ _ _ _ _ _ _ TRUE] -> w314
          tunnel: w308 -> [_ _ _ _ w360 _ _ _ _ _]
          tunnel: w312 -> [_ _ _ _ _ _ _ _ _ w420]
          frame Default {
            # "'Default' case only runs if there is a message that isn't defined in any of the other cases.  Output a programming error."
            n111 = Format Into String(format string="The invalid message string \"%s\" was received in the Message Handling Loop." ("Unknown Message Error Text"), w322) -> (resulting string=w320:string)  [unwired: 2 in, 1 out]
            n112 = call <vilib>:"Error Cluster From Error Code.vi"("error message (\"\")"=w320, "error code (0)"=1) -> ("error out"=w318:errorcluster)  [unwired: 7 in]
            n113 = Merge Errors(w318, w319) -> (w317:errorcluster)
          }
          frame "Initialize" {
            # "Initialize - Send separate messages to initialize the data and the front panel.  Bundle control references."
            n114 = control-ref of="Define Mask"() -> (w336:refnum<vi>)
            n115 = control-ref of="Stop"() -> (w334:refnum<vi>)
            n116 = control-ref of="Status Update"() -> (w335:refnum<vi>)
            n117 = control-ref of="Acquire Image"() -> (w337:refnum<vi>)
            n118 = call "IMAQ Create"("Image Name"="FPGA Image", "error in (no error)"=w327) -> ("New Image"=w332:T1, "error out"=w328:errorcluster)  [unwired: 3 in]
            n119 = call "IMAQ Create"("Image Name"="Processed Image", "error in (no error)"=w327) -> ("New Image"=w325:T1, "error out"=w326:errorcluster)  [unwired: 3 in]
            n120 = Bundle By Name(cluster=w339, "Acquire Image Ref"=w337, "Define Mask Ref"=w336, "Status Update Ref"=w335, "Stop Button Ref"=w334, "FPGA Image"=w332, "Processed Image"=w325) -> (w338:T16)
            n121 = call "Enqueue Message.vi"("error in (no error)"=w327, "Message"="Initialize Data", "Message Queue"=w342) -> ("error out"=w344:errorcluster, "dup Message Queue"=w343:refnum<queue>)  [unwired: 7 in]
            n122 = call "Enqueue Message.vi"("error in (no error)"=w344, "Message"="Initialize Panel", "Message Queue"=w343) -> ("error out"=w330:errorcluster)  [unwired: 7 in, 1 out]
            n123 = Merge Errors(w328, w326, w330) -> (w329:errorcluster)
          }
          frame "Initialize Data" {
            n124 = Bundle By Name(cluster=w348, "Initial Message"="Data Initialized") -> (w347:T16)
            n125 = Merge Errors(w349) -> (w345:errorcluster)
          }
          frame "Initialize Panel" {
            # "Code Needed - Initialize the appearance of the front panel"
            n126 = Unbundle By Name(w356) -> ("Initial Message"=w350:string)
            n127 = call "Enqueue Message.vi"("error in (no error)"=w354, "Message Data"=w350, "Message"="Update Display", "Message Queue"=w353) -> ("error out"=w352:errorcluster)  [unwired: 6 in, 1 out]
            n128 = Merge Errors(w352) -> (w355:errorcluster)
          }
          frame "Update Display" {
            # "Code Recommended - If you wish to decouple the Message Handling Loop from your user interface, consider creating User Events (like the \"Stop\" event in this VI) to message the Event Handling Loop whenever the user interface needs updating."
            # "Update Display - Convert the message data to a string to display in the  Status Update indicator."
            n129 = Variant To Data(error in=w361, type="", Variant=w360) -> (data=w357:string, error out=w358:errorcluster)
            n130 = Merge Errors(w358) -> (w362:errorcluster)
          }
          frame "Acquire Image" {
            # "This case acquires an image or stream from the FPGA frame grabber and displays on the front panel"
            n131 = while {
              tunnel: [w375] -> w364
              stop <- FALSE continue-if-true
              n132 = control-ref of="FPGA Image"() -> (w374:refnum<vi>)
              n133 = call "FPGA Frame Grabbing (Host).vi"("Ctl Refnum"=w374) -> ("Image"=w375:T1)
            }
            n134 = call "Enqueue Message.vi"("error in (no error)"=w365, "Message Data"="Image Acquired" ("\"Do Something\" button pressed"), "Message"="Update Display", "Message Queue"=w370) -> ("error out"=w371:errorcluster)  [unwired: 6 in, 1 out]
            n135 = Bundle By Name(cluster=w367, "FPGA Image"=w364) -> (w366:T16)
            n136 = Merge Errors(w371) -> (w372:errorcluster)
          }
          frame "Test FPGA" {
            # "This case sends mask parameters to the controls on the FPGA, then checks the extracted wingbeat signal"
            n137 = Unbundle By Name(w391) -> ("Left Annulus"=w390:T18, "Right Annulus"=w389:T18)
            n138 = Unbundle By Name(w390) -> ("Center X"=w387:i32, "Center Y"=w386:i32, "Inner Radius"=w383:i32, "Outer Radius"=w382:i32, "Start Angle"=w385:dbl, "End Angle"=w384:dbl)
            n139 = Unbundle By Name(w389) -> ("Center X"=w381:i32, "Center Y"=w380:i32, "Start Angle"=w379:dbl, "End Angle"=w378:dbl)
            n140 = local write "Status Update"("Testing FPGA Wingbeat Signals" ("Status Update")) -> ()
            n141 = Bundle By Name(cluster="Wing ROIs", "Left Hinge X"=w387, "Left Hinge Y"=w386, "Left Start Angle"=w385, "Left End Angle"=w384, "Inner Radius"=w383, "Outter Radius"=w382, "Right Hinge X"=w381, "Right Hinge Y"=w380, "Right Start Angle"=w379, "Right End Angle"=w378) -> (w377:T3)
            n142 = call "Enqueue Message.vi"("error in (no error)"=w394, "Message Data"="FPGA signal acquired" ("\"Do Something\" button pressed"), "Message"="Update Display", "Message Queue"=w393) -> ("error out"=w397:errorcluster)  [unwired: 6 in, 1 out]
            n143 = Merge Errors(w397) -> (w392:errorcluster)
            n144 = call "Wingbeat Amplitude Extraction (Host).vi"("Wing ROIs"=w377) -> ()  [unwired: 1 in]
            n145 = while {
              stop <- "Stop Charts" stop-if-true
              n146 = call "DAQ Assistant"() -> ("data"=w398:dynamicdata)  [unwired: 17 in, 2 out]
            }
          }
          frame "Test Visual Response" {
            # "This case starts a visual stimulation experiment to present patterns on the LED arena and record wingbeat signal in either open or closed loop. It analyzes the wingbeat response to visual stimulation to evaluate if the Wingbeat Analyzer is working properly."
            n147 = call "Enqueue Message.vi"("error in (no error)"=w402, "Message Data"="Tested Visual Response" ("\"Do Something\" button pressed"), "Message"="Update Display", "Message Queue"=w401) -> ("error out"=w405:errorcluster)  [unwired: 6 in, 1 out]
            n148 = Merge Errors(w405) -> (w400:errorcluster)
          }
          frame "Save Mask" {
            # "This case saves the current mask parameters to disk so other VIs can use them to control the FPGA"
            n149 = call "Enqueue Message.vi"("error in (no error)"=w407, "Message Data"="Mask parameters saved" ("\"Do Something Else\" button pressed"), "Message"="Update Display", "Message Queue"=w409) -> ("error out"=w408:errorcluster)  [unwired: 6 in, 1 out]
            n150 = Merge Errors(w408) -> (w412:errorcluster)
          }
          frame "Exit" {
            # "Stop the VI"
            # "Release the message queue reference"
            # "Code Needed - Add any required cleanup code here"
            n151 = call "Fire User Event - Stop.vi"("User Event - Stop"=w420) -> ("error out"=w419:errorcluster)  [unwired: 10 in]
            n152 = Release Queue(queue=w425, error in (no error)=w414) -> (error out=w422:errorcluster)  [unwired: 1 in, 2 out]
            n153 = call "IMAQ WindClose"("Close All Windows (False)"=TRUE, "error in (no error)"=w414) -> ("error out"=w416:errorcluster)  [unwired: 4 in]
            n154 = call "IMAQ Dispose"("All Images? (No)"=TRUE, "error in (no error)"=w416) -> ("error out"=w415:errorcluster)  [unwired: 4 in]
            n155 = Merge Errors(w415, w419, w422) -> (w421:errorcluster)
          }
        }
      }
      n156 = while {
        tunnel: w244 -> [w254]
        tunnel: [w250] -> w237
        shift-right: [w248] -> w236
        shift-left: w243 -> [w249]
        tunnel: w234 -> [w247]
        stop <- w252 stop-if-true
        # "Event Handling Loop"
        n157 = event shown="[2] \"Test FPGA\": Value Change" {
          selector: w249 -> [_ _ _ _ _ _ _ _]
          dyn-events: [_ _ _ _ _ _ _ _] -> w248
          timeout: _ -> [_ _ _ _ _ _ _ _]
          tunnel: [FALSE ("Discard?") FALSE ("Discard?") FALSE ("Discard?") FALSE ("Discard?") FALSE ("Discard?") w296 FALSE ("Discard?") TRUE ("Discard?")] -> w253
          tunnel: w254 -> [w265 w271 w277 w282 w287 w295 w302 w305]
          tunnel: [w264 w269 w274 w279 w284 w294 w301 _] -> w250
          tunnel: [w263 w270 w273 w281 w286 w293 w299 w305] -> w251
          tunnel: w247 -> [w261 w267 w275 w278 w285 w290 _ _]
          event "Acquire Image": Value Change {
            n158 = event-data() -> ()  [unwired: 1 in, 1 out]
            n159 = call "Enqueue Message.vi"("error in (no error)"=w261, "Message"="Acquire Image", "Message Queue"=w265) -> ("error out"=w264:errorcluster, "dup Message Queue"=w263:refnum<queue>)  [unwired: 7 in]
          }
          event "Define Mask": Value Change {
            n160 = event-data() -> ()  [unwired: 1 in, 1 out]
            n161 = call "Enqueue Message.vi"("error in (no error)"=w267, "Message"="Define Mask", "Message Queue"=w271) -> ("error out"=w269:errorcluster, "dup Message Queue"=w270:refnum<queue>)  [unwired: 7 in]
          }
          event "Test FPGA": Value Change {
            n162 = event-data() -> ()  [unwired: 1 in, 1 out]
            n163 = call "Enqueue Message.vi"("error in (no error)"=w275, "Message"="Test FPGA", "Message Queue"=w277) -> ("error out"=w274:errorcluster, "dup Message Queue"=w273:refnum<queue>)  [unwired: 7 in]
          }
          event "Test Visual Response": Value Change {
            n164 = event-data() -> ()  [unwired: 1 in, 1 out]
            n165 = call "Enqueue Message.vi"("error in (no error)"=w278, "Message"="Test Visual Response", "Message Queue"=w282) -> ("error out"=w279:errorcluster, "dup Message Queue"=w281:refnum<queue>)  [unwired: 7 in]
          }
          event #4 (no event record) {
            n166 = event-data() -> ()  [unwired: 1 in, 1 out]
            n167 = call "Enqueue Message.vi"("error in (no error)"=w285, "Message"="Save Mask", "Message Queue"=w287) -> ("error out"=w284:errorcluster, "dup Message Queue"=w286:refnum<queue>)  [unwired: 7 in]
          }
          event Panel Close? {
            w296 = TRUE ("Discard?")
            n168 = event-data() -> ()  [unwired: 1 in, 1 out]
            n169 = call "Enqueue Message.vi"("Priority Message? (F)"=TRUE, "error in (no error)"=w290, "Message"="Exit", "Message Queue"=w295) -> ("error out"=w294:errorcluster, "dup Message Queue"=w293:refnum<queue>)  [unwired: 6 in]
            n170 = event-data("Discard?"=w296) -> ()  [unwired: 1 in, 1 out]
          }
          event "Stop": Value Change {
            n171 = event-data() -> ()  [unwired: 1 in, 1 out]
            n172 = call "Enqueue Message.vi"("Priority Message? (F)"=TRUE, "Message"="Exit", "Message Queue"=w302) -> ("error out"=w301:errorcluster, "dup Message Queue"=w299:refnum<queue>)  [unwired: 7 in]
          }
          event User Event {
            # "The Message Handling Loop processed an \"Exit\" message, which fired this event to stop the Event Handling Loop."
            n173 = event-data() -> ()  [unwired: 1 in, 1 out]
            n174 = local write "Status Update"("VI Stopped" ("VI Stopped")) -> ()
          }
        }
        n175 = case shown="No Error" w250 {
          tunnel: [w255 TRUE ("Discard?")] -> w252
          tunnel: w253 -> [w255 _]
          tunnel: w251 -> [_ w258]
          frame No Error {
          }
          frame Error {
            # "On error, send Exit message, and stop loop."
            n176 = call "Enqueue Message.vi"("Priority Message? (F)"=TRUE, "Message"="Exit", "Message Queue"=w258) -> ()  [unwired: 7 in, 2 out]
          }
        }
      }
      n177 = Unregister For Events(event registration refnum=w236, error in=w237) -> (error out=w238:errorcluster)
      n178 = Merge Errors(w238, w245) -> (w240:errorcluster)
      n179 = call "Destroy User Event - Stop.vi"("error in (no error)"=w240, "User Event - Stop"=w239) -> ("error out"=w241:errorcluster)  [unwired: 9 in]
      n180 = call <vilib>:"Simple Error Handler.vi"("error in (no error)"=w241) -> ()  [unwired: 4 in, 5 out]
    }
    frame Enabled {
    }
  }
